vi "CSE ISP - vc menu item properties.vi"(6 "error in":errorcluster, 9 "ISP menu":refnum<k9>) -> (0 "error out":errorcluster, 3 "dup ISP menu":refnum<k9>)   [LabVIEW 2021]
doc: "::: CalcExpress Toolkit :::\nCopyright (c) 2000-2026 Konstantin Shifershteyn. All rights reserved."
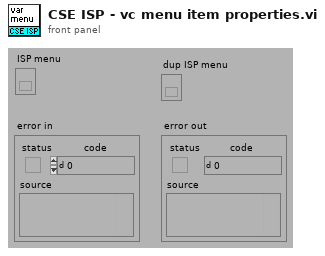
[diagram p1: front panel]
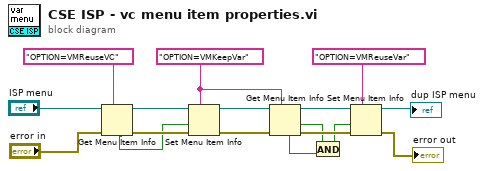
[diagram p0: block diagram]
diagram:
  w13 = "OPTION=VMKeepVar" ("item tag")
  n1 = Get Menu Item Info(7:"OPTION=VMReuseVC" ("item tag"), 8:"error in", 11:"ISP menu") -> (0:w10:errorcluster, 3:w11:refnum<k9>, 4:w5:bool)  [unwired: 4 out]
  n2 = Set Menu Item Info(7:w13, 8:w10, 9:w5, 11:w11) -> (0:w9:errorcluster, 3:w12:refnum<k9>)  [unwired: 3 in]
  n3 = Get Menu Item Info(7:w13, 8:w9, 11:w12) -> (0:w15:errorcluster, 1:w8:bool, 3:w16:refnum<k9>, 4:w7:bool)  [unwired: 3 out]
  n4 = And(x=w8, y=w7) -> (x .and. y?=w6:bool)
  n5 = Set Menu Item Info(7:"OPTION=VMReuseVar" ("item tag"), 8:w15, 9:w6, 11:w16) -> (0:→"error out":errorcluster, 3:→"dup ISP menu":refnum<k9>)  [unwired: 3 in]
